vi "VM Spy - build list of contexts.vi"(7 "sort column":i32(ring) items=["handle", "name"], 9 "MCListbox Refnum":refnum<vi>) -> (1 "updated":bool, 2 "array of VC handles":T1[](array[typedef]), 3 "dup MCListbox Refnum":refnum<vi>)   [LabVIEW 2021]
doc: "::: CalcExpress Toolkit :::\nCopyright (c) 2000-2026 Konstantin Shifershteyn. All rights reserved."
uses:
  vi.lib/addons/CalcExpress/cetypes.llb/VarMan Variable Context Handle.ctl
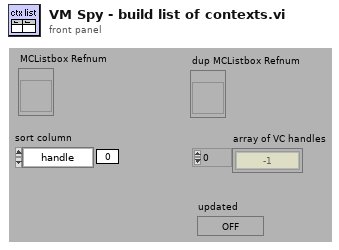
[diagram p1: front panel]
types:
  T1 = typedef "VarMan Variable Context Handle.ctl" = i32
  T2 = enum32{"nothing", "reset", "assign name", "get name", "get handle"}
  T3 = cluster{"VC Handle out":T1, "VC Name out":string}
  T4 = cluster{"VC Handle out":T1, "VC Name out":string}[]
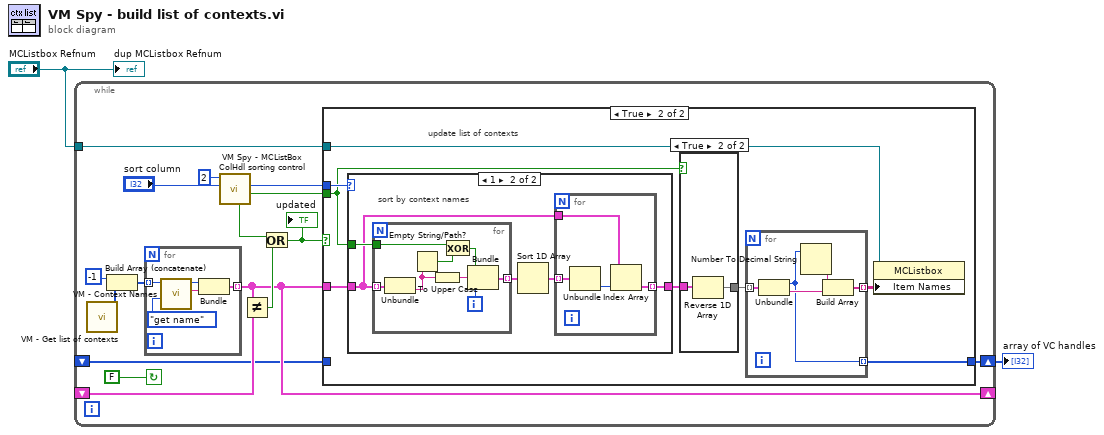
[diagram p0: block diagram]
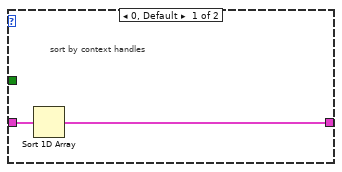
[diagram p4: hidden frame]
diagram:
  n1 = while {
    shift-right: [w9] -> _
    shift-left: _ -> [w13]
    shift-right: [w8] -> w2
    shift-left: _ -> [w7]
    tunnel: "MCListbox Refnum" -> [w5]
    stop <- FALSE continue-if-true
    n2 = call "VM - Get list of contexts.vi"() -> ("array of VC handles"=w17:T1[])  [unwired: 7 in, 2 out]
    n3 = Build Array (concatenate)(T1 -1 ("VC Handle"), w17) -> (w15:T1[])
    n4 = for {
      tunnel: w15 -> [w58] mode=indexing
      tunnel: [w55] -> w9 mode=indexing
      n5 = call "VM - Context Names.vi"("action"=T2."get name", "VC Handle"=w58) -> ("VC Name out"=w56:string, "VC Handle out"=w57:T1)  [unwired: 4 in, 2 out]
      n6 = Bundle("VC Handle out"=w57, "VC Name out"=w56) -> (w55:T3)  [unwired: 1 in]
    }
    n7 = call "VM Spy - MCListBox ColHdl sorting control.vi"("sort column"="sort column", "Total columns"=2) -> ("reversed order"=w10:bool, "column to sort"=w11:i32, "update required"=w14:bool)  [unwired: 7 in]
    n8 = Not Equal?(x=w9, y=w13) -> (x != y?=w12:bool)
    n9 = Or(x=w14, y=w12) -> (x .or. y?=w4:bool)
    "updated" <- w4
    n10 = case shown="True" w4 {
      tunnel: w11 -> [_ w27]
      tunnel: w10 -> [_ w24]
      tunnel: w9 -> [_ w26]
      tunnel: w5 -> [_ w21]
      tunnel: [w19 w20] -> w8
      tunnel: w7 -> [w19 _]
      frame False {
        # "nothing changed"
      }
      frame True {
        # "update list of contexts"
        n11 = case shown="1" w27 {
          tunnel: w26 -> [w37 w39]
          tunnel: [w36 w38] -> w25
          tunnel: w24 -> [_ w42]
          frame 0, Default {
            # "sort by context handles"
            n12 = Sort 1D Array(array=w37) -> (sorted array=w36:T4)
          }
          frame 1 {
            # "sort by context names"
            n13 = for {
              tunnel: w39 -> [w54] mode=indexing
              tunnel: w42 -> [w49]
              tunnel: [w48] -> w41 mode=indexing
              i -> [w47]
              n14 = Unbundle(w54) -> ("VC Name out"=w50:string)  [unwired: 1 out]
              n15 = Empty String/Path?(string/path=w50) -> (empty?=w52:bool)
              n16 = To Upper Case(1:w50) -> (0:w51:string)
              n17 = Exclusive Or(1:w52, 2:w49) -> (0:w53:bool)
              n18 = Bundle(w53, w51, w47) -> (w48:cluster{bool, string, i32})  [unwired: 1 in]
            }
            n19 = Sort 1D Array(array=w41) -> (sorted array=w40:cluster{bool, string, i32}[])
            n20 = for {
              tunnel: w40 -> [w46] mode=indexing
              tunnel: w39 -> [w44]
              tunnel: [w43] -> w38 mode=indexing
              n21 = Unbundle(w46) -> (w45:i32)  [unwired: 2 out]
              n22 = Index Array(array=w44, index=w45) -> (element=w43:T3)
            }
          }
        }
        n23 = case shown="True" w24 {
          tunnel: w25 -> [w33 w35]
          tunnel: [w33 w34] -> w23
          frame False {
          }
          frame True {
            n24 = Reverse 1D Array(array=w35) -> (reversed array=w34:T4)
          }
        }
        n25 = for {
          tunnel: w23 -> [w32] mode=indexing
          tunnel: [w29] -> w22 mode=indexing
          tunnel: [w28] -> w20 mode=indexing
          n26 = Unbundle(w32) -> ("VC Handle out"=w28:T1, "VC Name out"=w30:string)
          n27 = Number To Decimal String(number=w28) -> (decimal integer string=w31:string)  [unwired: 1 in]
          n28 = Build Array(w31, w30) -> (w29:string[])
        }
        n29 = property on="Property Node" class="MCListbox"(reference=w21, "Item Names"=w22) -> ()  [unwired: 1 in, 2 out]
      }
    }
  }
  "array of VC handles" <- w2
  "dup MCListbox Refnum" <- "MCListbox Refnum"
